vi "Test Decode JSON.vi"(8 "error in (no error)":errorcluster) -> (0 "error out":errorcluster)   [LabVIEW 2019]
uses:
  58e0d79b-ccb6-498d-8073-75b35f77733f.vi
  58e0d79b-ccb6-498d-8073-75b35f77733f.vi/c2cf74e5-7d8b-40fb-bd29-b538da81d03b.vi
  58e0d79b-ccb6-498d-8073-75b35f77733f.vi/fd9e35e6-15e9-47e7-b0f6-24f1efe1d84e.vi
  <vilib>/Utility/Data Type/Get Type Information.vi
  <vilib>/JDP Science/JSONtext/JSON text to Variant.vi
  <vilib>/JDP Science/JSONtext/LVClass Serializer/JSONtext LVClass Serializer.lvclass
  <userlib>/LevyLab/JSON-RPC/JSON-RPC.lvlib
  <vilib>/addons/_JKI Toolkits/Caraya/classes/Assert/Assert.lvclass
  <vilib>/addons/_JKI Toolkits/Caraya/classes/Test/Test.lvclass
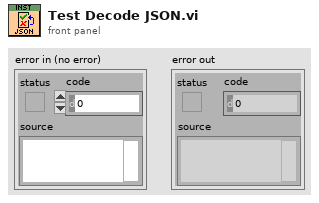
[diagram p1: front panel]
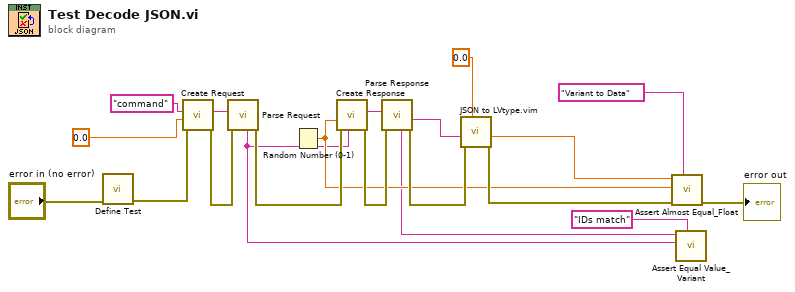
[diagram p0: block diagram]
diagram:
  n1 = call <vilib>:"Define Test.vi"("error in (no error)"="error in (no error)") -> ("error out"=w15:errorcluster)  [unwired: 9 in, 1 out]
  n2 = call <userlib>:"Create Request.vi"("error in (no error)"=w15, "params"=0.0, "method"="command") -> ("error out"=w16:errorcluster, "<JSON> Requests"=w20:string)  [unwired: 6 in, 1 out]
  n3 = call <userlib>:"Parse Request.vi"("error in (no error)"=w16, "<JSON> Requests"=w20) -> ("error out"=w17:errorcluster, "IDs"=w2:string)  [unwired: 6 in, 2 out]
  n4 = Random Number (0-1)() -> (number: 0 to 1=w4:dbl)
  n5 = call <userlib>:"Create Response.vi"("id"=w2, "error in (no error)"=w17, "result"=w4) -> ("error out"=w18:errorcluster, "<JSON> Response"=w19:string)  [unwired: 7 in]
  n6 = call <userlib>:"Parse Response.vi"("error in (no error)"=w18, "<JSON> Response"=w19) -> ("error out"=w8:errorcluster, "results"=w10:string, "IDs"=w3:string)  [unwired: 7 in]
  n7 = call "JSON to LVtype.vim"("type"=0.0, "error in (no error)"=w8, "JSON Data in"=w10) -> ("error out"=w7:errorcluster, "Data out"=w9:dbl)  [unwired: 7 in]
  n8 = call <vilib>:"Assert Almost Equal_Float.vi"("Label"="Variant to Data", "error in (no error)"=w7, "Y"=w4, "X"=w9) -> ("error out"=→"error out":errorcluster)  [unwired: 6 in, 1 out]
  n9 = call <vilib>:"Assert Equal Value_Variant.vi"("Label"="IDs match", "Y"=w2, "X"=w3) -> ()  [unwired: 7 in, 2 out]
